vi "Item_OnCommand.vi"(10 "Command ID":string, 11 "Object":T1) -> ()   [LabVIEW 2020, in "Project Provider.lvlib"]
uses:
  Project Provider.lvlib
  <resource>/Framework/Providers/API/ItemRef.ctl
  <vilib>/Utility/error.llb/Error Cluster From Error Code.vi
  <vilib>/ErrorRing/Error Ring.xnode
panel:
  out "error out":errorcluster
  in  "error in":errorcluster
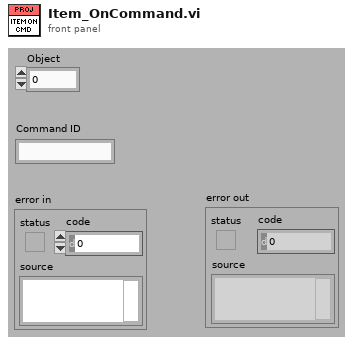
[diagram p1: front panel]
types:
  T1 = typedef "ItemRef.ctl" = u64
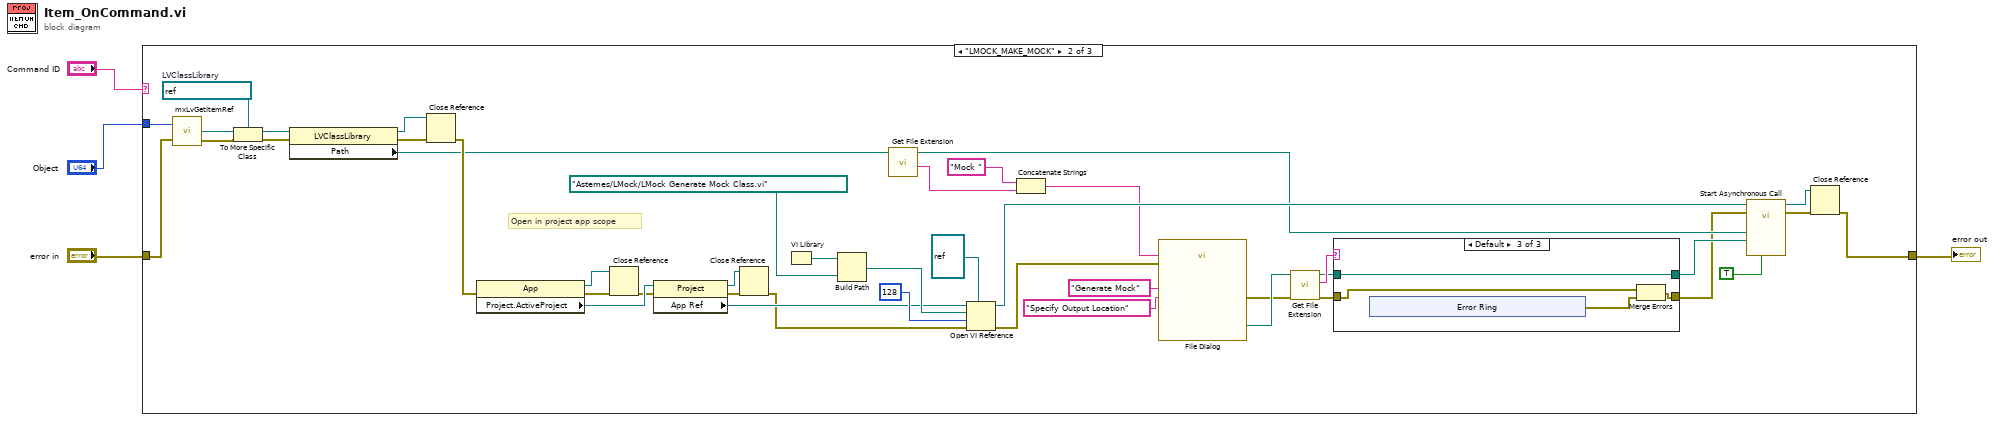
[diagram p0: block diagram]
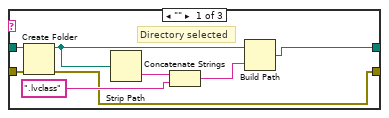
[diagram p3: hidden frame]
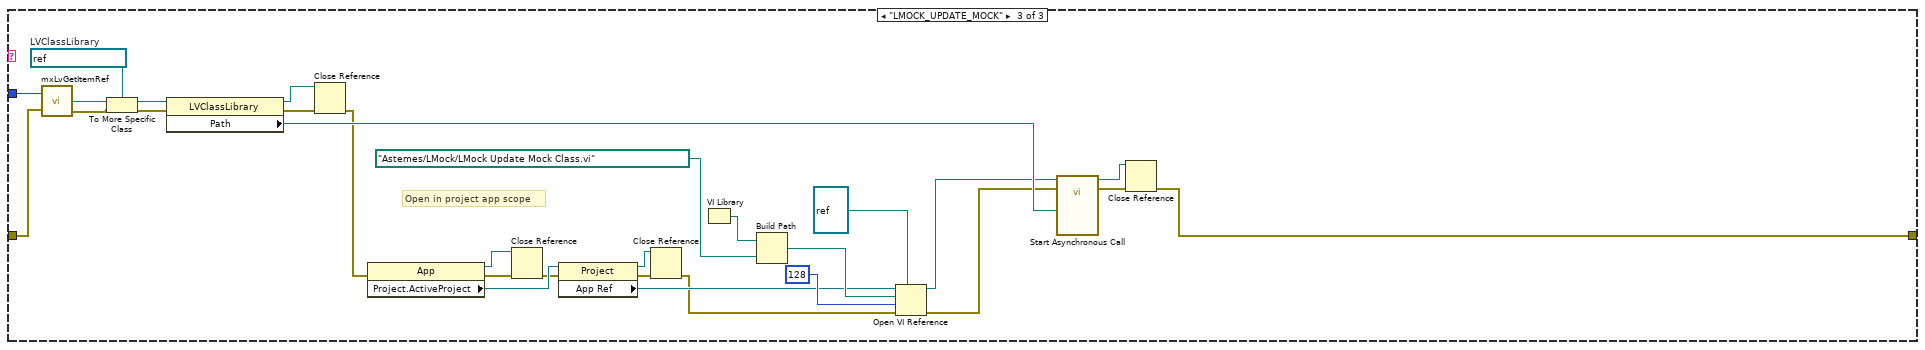
[diagram p5: hidden frame]
diagram:
  n1 = case shown="\"LMOCK_MAKE_MOCK\"" "Command ID" {
    tunnel: "error in" -> [w5 w47 w94]
    tunnel: [w5 w23 w70] -> w2
    tunnel: "Object" -> [_ w48 w95]
    frame Default {
    }
    frame "LMOCK_MAKE_MOCK" {
      w44 = refnum<vi> refnum  # LVClassLibrary
      # "Open in project app scope"
      n2 = call <resource>:"mxLvGetItemRef.vi"("Item"=w48, "error in"=w47) -> ("Item Refnum"=w46:refnum<vi>, "error out"=w38:errorcluster)  [unwired: 1 out]
      n3 = To More Specific Class(target class=w44, reference=w46, error in=w38) -> (specific class reference=w45:refnum<vi>, error out=w43:errorcluster)
      n4 = property class="LVClassLibrary"(reference=w45, error in=w43) -> (reference out=w41:refnum<vi>, error out=w42:errorcluster, "Path"=w14:path)
      n5 = Close Reference(reference=w41, error in (no error)=w42) -> (error out=w34:errorcluster)
      n6 = property class="App"(error in=w34) -> (reference out=w24:refnum<vi>, error out=w26:errorcluster, "Project.ActiveProject"=w31:refnum<vi>)  [unwired: 1 in]
      n7 = Close Reference(reference=w24, error in (no error)=w26) -> (error out=w25:errorcluster)
      n8 = property class="Project"(reference=w31, error in=w25) -> (reference out=w30:refnum<vi>, error out=w28:errorcluster, "App Ref"=w29:refnum<vi>)
      n9 = Close Reference(reference=w30, error in (no error)=w28) -> (error out=w27:errorcluster)
      n10 = VI Library() -> (path=w32:path)
      n11 = Build Path(base path=w32, name or relative path=path "Astemes/LMock/LMock Generate Mock Class.vi" ("Relative Path from 1 to 2")) -> (appended path=w37:path)
      n12 = call <vilib>:"Get File Extension.vi"("file"=w14) -> ("filename without extension"=w15:string, "dup file"=w13:path)  [unwired: 6 in, 3 out]
      n13 = Open VI Reference(type specifier VI Refnum (for type only)=refnum<vi> refnum, application reference (local)=w29, vi path=w37, options=128, error in (no error)=w27) -> (vi reference=w36:refnum<vi>, error out=w20:errorcluster)  [unwired: 1 in]
      n14 = Concatenate Strings("Mock " ("string"), w15) -> (w17:string)
      n15 = call "File Dialog"("prompt"="Specify Output Location", "button label"="Generate Mock", "default name"=w17, "error in"=w20) -> ("selected path"=w9:path, "error out"=w6:errorcluster)  [unwired: 8 in, 2 out]
      n16 = call <vilib>:"Get File Extension.vi"("error in (no error)"=w6, "file"=w9) -> ("error out"=w12:errorcluster, "lowercase file extension"=w11:string, "dup file"=w10:path)  [unwired: 5 in, 2 out]
      n17 = case shown="Default" w11 {
        tunnel: w12 -> [w54 w57 w59]
        tunnel: w10 -> [w52 w58 w61]
        tunnel: [w53 w57 w60] -> w7
        tunnel: [w49 w58 w61] -> w8
        frame "" {
          # "Directory selected"
          n18 = Create Folder(path (use dialog)=w52, error in=w54) -> (created path=w50:path, error out=w53:errorcluster)  [unwired: 1 in, 1 out]
          n19 = Strip Path(path=w50) -> (name=w56:string)  [unwired: 1 out]
          n20 = Concatenate Strings(w56, ".lvclass" ("string")) -> (w51:string)
          n21 = Build Path(base path=w50, name or relative path=w51) -> (appended path=w49:path)
        }
        frame "lvclass" {
        }
        frame Default {
          n22 = xnode "Error Ring"() -> ("error out"=w62:errorcluster)
          n23 = Merge Errors(w59, w62) -> (w60:errorcluster)
        }
      }
      n24 = call-by-ref "Start Asynchronous Call"(reference=w36, error in=w7, "Add to lvproj?"=TRUE, "Destination Class Path"=w8, "Source Class Path"=w13) -> (reference out=w39:refnum<vi>, error out=w40:errorcluster)  [unwired: 7 in, 2 out]
      n25 = Close Reference(reference=w39, error in (no error)=w40) -> (error out=w23:errorcluster)
    }
    frame "LMOCK_UPDATE_MOCK" {
      w91 = refnum<vi> refnum  # LVClassLibrary
      # "Open in project app scope"
      n26 = call <resource>:"mxLvGetItemRef.vi"("Item"=w95, "error in"=w94) -> ("Item Refnum"=w93:refnum<vi>, "error out"=w84:errorcluster)  [unwired: 1 out]
      n27 = To More Specific Class(target class=w91, reference=w93, error in=w84) -> (specific class reference=w92:refnum<vi>, error out=w90:errorcluster)
      n28 = property class="LVClassLibrary"(reference=w92, error in=w90) -> (reference out=w88:refnum<vi>, error out=w89:errorcluster, "Path"=w86:path)
      n29 = Close Reference(reference=w88, error in (no error)=w89) -> (error out=w80:errorcluster)
      n30 = property class="App"(error in=w80) -> (reference out=w71:refnum<vi>, error out=w73:errorcluster, "Project.ActiveProject"=w78:refnum<vi>)  [unwired: 1 in]
      n31 = Close Reference(reference=w71, error in (no error)=w73) -> (error out=w72:errorcluster)
      n32 = property class="Project"(reference=w78, error in=w72) -> (reference out=w77:refnum<vi>, error out=w75:errorcluster, "App Ref"=w76:refnum<vi>)
      n33 = Close Reference(reference=w77, error in (no error)=w75) -> (error out=w74:errorcluster)
      n34 = VI Library() -> (path=w67:path)
      n35 = Build Path(base path=w67, name or relative path=path "Astemes/LMock/LMock Update Mock Class.vi" ("Relative Path from 1 to 2")) -> (appended path=w83:path)
      n36 = Open VI Reference(type specifier VI Refnum (for type only)=refnum<vi> refnum, application reference (local)=w76, vi path=w83, options=128, error in (no error)=w74) -> (vi reference=w82:refnum<vi>, error out=w69:errorcluster)  [unwired: 1 in]
      n37 = call-by-ref "Start Asynchronous Call"(reference=w82, error in=w69, "Source Class Path"=w86) -> (reference out=w85:refnum<vi>, error out=w87:errorcluster)  [unwired: 10 in, 1 out]
      n38 = Close Reference(reference=w85, error in (no error)=w87) -> (error out=w70:errorcluster)
    }
  }
  "error out" <- w2
